vi "recall Preset File.vi"(8 "error in (no error)":errorcluster caption="에러 입력(에러 없음)", 10 "File Path":string, 11 "FSV-40N 입력":refnum<class "FSV-40N.lvclass">) -> (0 "error out":errorcluster caption="에러 출력", 3 "FSV-40N 출력":refnum<class "FSV-40N.lvclass">)   [LabVIEW 2023, in "Spectrum Analyzer.lvlib" / "FSV-40N.lvclass"]
uses:
  FSV-40N.lvclass
  FSV-40N.lvclass/FSV-40N.ctl
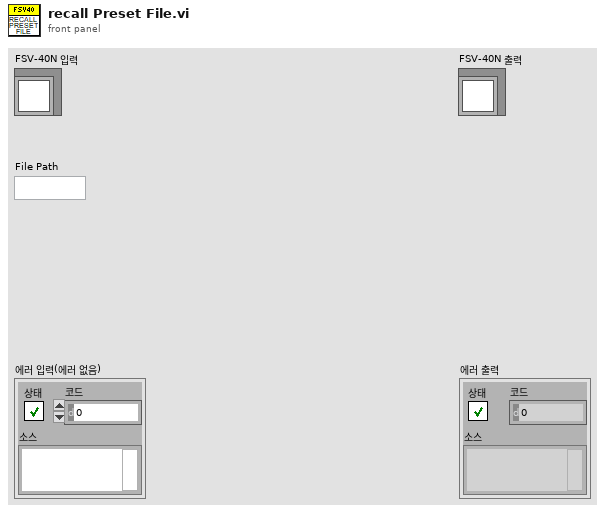
[diagram p1: front panel]
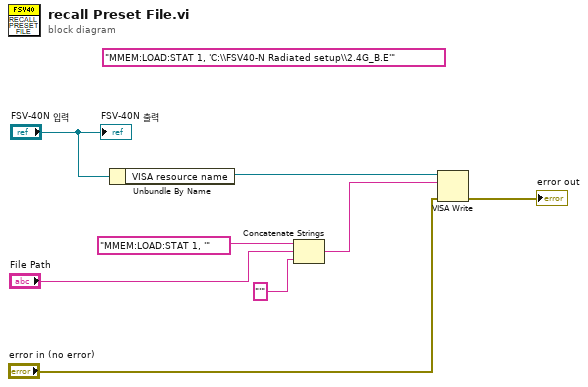
[diagram p0: block diagram]
diagram:
  (unwired) "MMEM:LOAD:STAT 1, 'C:\\FSV40-N Radiated setup\\2.4G_B.E'" ("write buffer")
  n1 = Unbundle By Name("FSV-40N 입력") -> ("VISA resource name"=w8:refnum<visa-resource-name>)
  n2 = Concatenate Strings("MMEM:LOAD:STAT 1, '" ("write buffer"), "File Path", "'" ("string")) -> (w5:string)
  n3 = VISA Write(VISA resource name=w8, write buffer=w5, error in (no error)="error in (no error)") -> (error out=→"error out":errorcluster)  [unwired: 2 out]
  "FSV-40N 출력" <- "FSV-40N 입력"
